vi "Measurement UI.vi"() -> ()   [LabVIEW 2022 SP3, in "Efficiency_Class D Amplifier_UI.lvlib"]
uses:
  Efficiency_Class D Amplifier_UI.lvlib
  shared/controls/units - snr.ctl
  shared/controls/units - ratio.ctl
  shared/controls/digital output level units.ctl
  shared/ui/controls/view.ctl
  shared/controls/power measurement method.ctl
  UI State.ctl
  <vilib>/Utility/miscctls.llb/LVBoundsTypeDef.ctl
  <vilib>/Utility/miscctls.llb/LVPoint32TypeDef.ctl
  <vilib>/Utility/miscctls.llb/LVPointTypeDef.ctl
  shared/ui/UI Helpers.lvlib
  shared/audio popup ui/Audio Popup UI.lvlib
  shared/controls/audio controls.lvlib
panel:
  in  "view legend":T1
  out "time domain":waveform(dbl)[](graph)
  out "frequency domain":cluster{"x0":dbl, "dx":dbl, "magnitude":dbl[]}[](graph)
  out "efficiency (%)":dbl caption="Efficiency" format="%#.2g%"
  out "power loss (W)":dbl caption="Power Loss" format="%#.2g W"
  out "total output power (W)":dbl caption="Total Output Power" format="%#.2g W"
  out "input power (W)":dbl caption="Input Power" format="%#.2g W"
  out "meas table":string[][](table)
  in  "digital serial cfg file":string
  in  "power measurement resource":string="PXI1Slot4/ai0"
  out "output power (W)":dbl[](array[numeric])
  out "SFDR (dBc)":dbl[](array[numeric])
  out "gain":dbl[](array[numeric])
  out "dynamic range (dB)":dbl[](array[numeric])
  out "THD":dbl[](array[numeric])
  out "THD+N":dbl[](array[numeric])
  out "SNR":dbl[](array[numeric])
  out "phase (deg)":dbl[](array[numeric])
  out "amplitude (dBFS)":dbl[](array[numeric])
  out "amplitude (Vrms)":dbl[](array[numeric])
  out "frequency (Hz)":dbl[](array[numeric])
  out "channel names":string[](array[string])
  in  "Configuration tab":enum32{"Protocol", "Measurement", "Units"}(tab)
  out "digital serial file name":string
  in  "configure digital serial":bool
  in  "master clock channel list":string caption="Master Clock Channel"
  in  "digital channel list":string caption="Digital Audio Channel"
  in  "sense resistor (Ohms)":dbl caption="Sense Resistor" format="%#_g Ohms"
  in  "power supply current limit":dbl caption="Current Limit" format="%#_g A"
  in  "power supply voltage":dbl caption="Power Supply Voltage" format="%#_g V"
  in  "power meas resource":refnum<k15> caption="Resource"
  in  "power measurement method":T2 caption="Method"
  in  "output level":dbl=-1.0 caption="Output level" format="%#_3f"
  in  "output level units":T3
  in  "min settling cycles":u32 caption="Minimum settling cycles"
  in  "min settling time (s)":dbl=0.1 caption="Minimum settling time" format="%#_6ps"
  in  "min measurement cycles":u32 caption="Minimum measurement cycles"
  in  "min measurement time (s)":dbl=0.1 caption="Minimum measurement time" format="%#_6ps"
  in  "Acquisition channel":tag
  in  "acq sampling rate":dbl=51200.0 caption="Sample rate" format="%#.6pHz"
  in  "lowpass filter":T4(ring) caption="Lowpass filter"
  in  "highpass filter":enum32{"DC", "AC"}(ring) caption="Highpass filter"
  in  "band start":dbl=20.0 caption="Band start" format="%#_6pHz"
  in  "band stop":dbl=20000.0 caption="Band stop" format="%#_6pHz"
  in  "weighting filter":T5(ring)=enum."A-weighting" caption="Weighting filter"
  in  "load impedance":dbl=4.0 caption="Load impedance" format="%#_6p Ohms"
  in  "output range (pk-pk)":dbl=15.0 caption="Output range" format="%.3p Vpk-pk"
  in  "signal frequency":dbl=1000.0 caption="Frequency" format="%#_6pHz"
  in  "gain units":T6 caption="Gain"
  in  "THD units":T6 caption="THD"
  in  "THD+N units":T6 caption="THD+N"
  in  "SNR units":T7 caption="SNR"
  in  "channel 0 offset":u32=1
  out "fft - data":dbl[](array[numeric])
  out "fft - df":dbl
  out "fft - f0":dbl
  out "wfm - data":dbl[](array[numeric])
  out "wfm - dt":dbl
  out "wfm - t0":dbl
  in  "acq channel":string="PXI1Slot4/ai0"
  in  "signal phase":dbl caption="phase"
  # "hidden controls - used to sync with MeasLink"
  # "hidden indicators"
  # "Digital Serial Settings"
  # "Harware Resource"
  # "Filters"
  # "Output"
  # "Acquisition"
  # "Power"
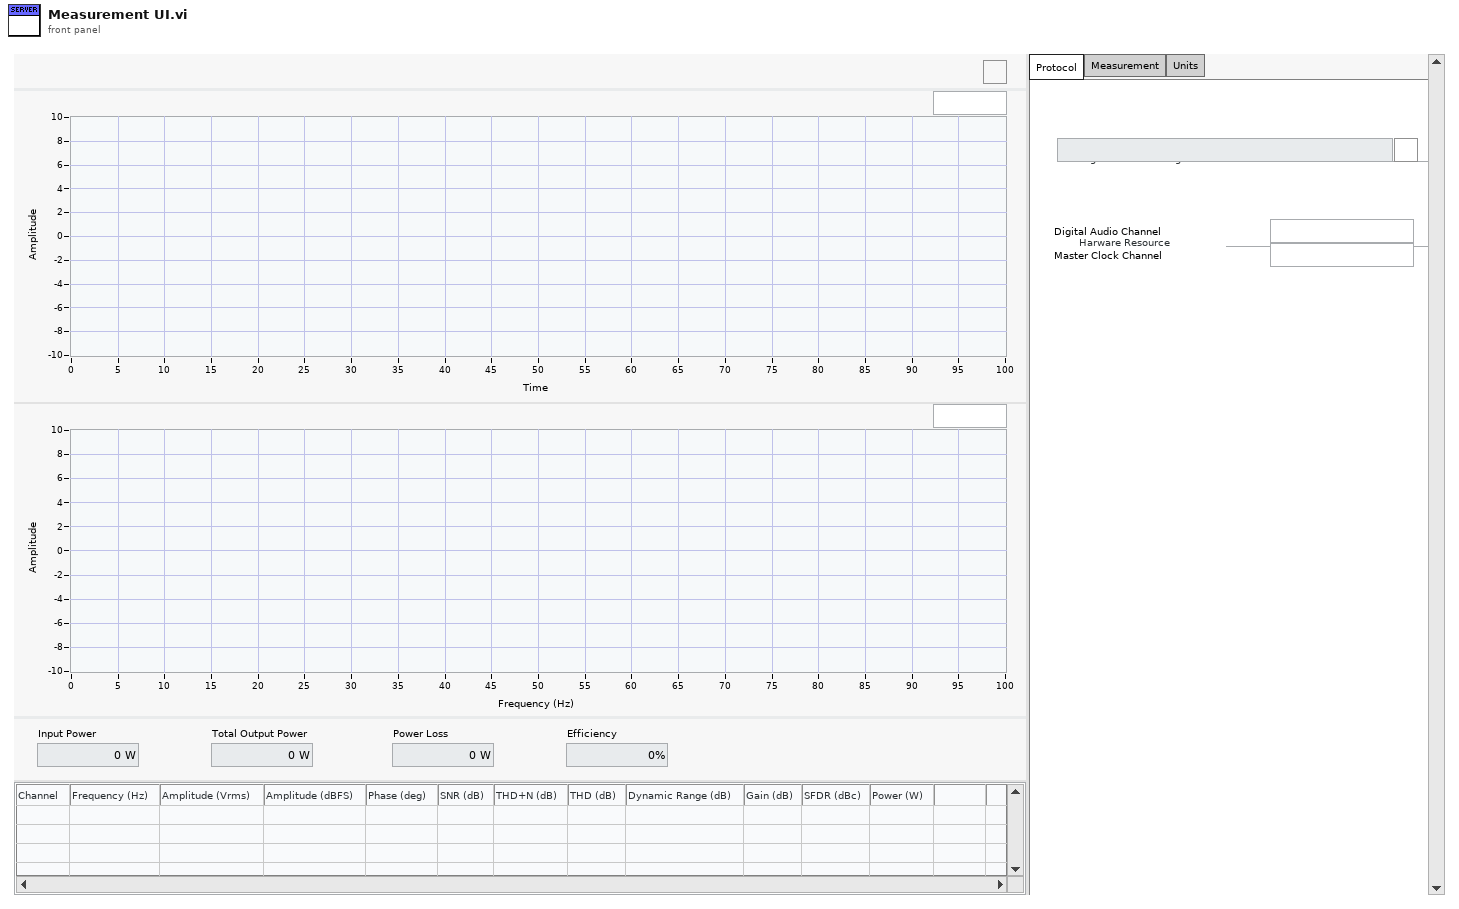
[diagram p1: front panel]
types:
  T1 = typedef "UI Helpers.lvlib/view.ctl" = bool
  T2 = typedef "power measurement method.ctl" = enum32{"SMU", "DMM"}
  T3 = typedef "audio controls.lvlib/digital output level units.ctl" = enum32{"% FS", "dBFS", "V"}
  T4 = enum32{"No filter", "AES17 20kHz", "AES17 40kHz"}
  T5 = enum32{"Linear", "A-weighting", "B-weighting", "C-weighting"}
  T6 = typedef "audio controls.lvlib/units - ratio.ctl" = enum32{"dB", "%", "x/y"}
  T7 = typedef "audio controls.lvlib/units - snr.ctl" = enum32{"dB", "x/y"}
  T8 = typedef "Efficiency_Class D Amplifier_UI.lvlib/UI State.ctl" = cluster{"Graph Size":T9, "Legend Visible":bool, "Mouse Coords":T10, "PostUI event occurred":bool, "digital serial cfg file":path}
  T9 = typedef "LVBoundsTypeDef.ctl" = cluster{"Width":u32, "Height":u32}
  T10 = typedef "LVPoint32TypeDef.ctl" = cluster{"Horizontal":i32, "Vertical":i32}
  T11 = typedef "LVPointTypeDef.ctl" = cluster{"Horizontal":i16, "Vertical":i16}
  T12 = typedef "Audio Popup UI.lvlib/audio settings.ctl" = cluster{"digital serial file":string}
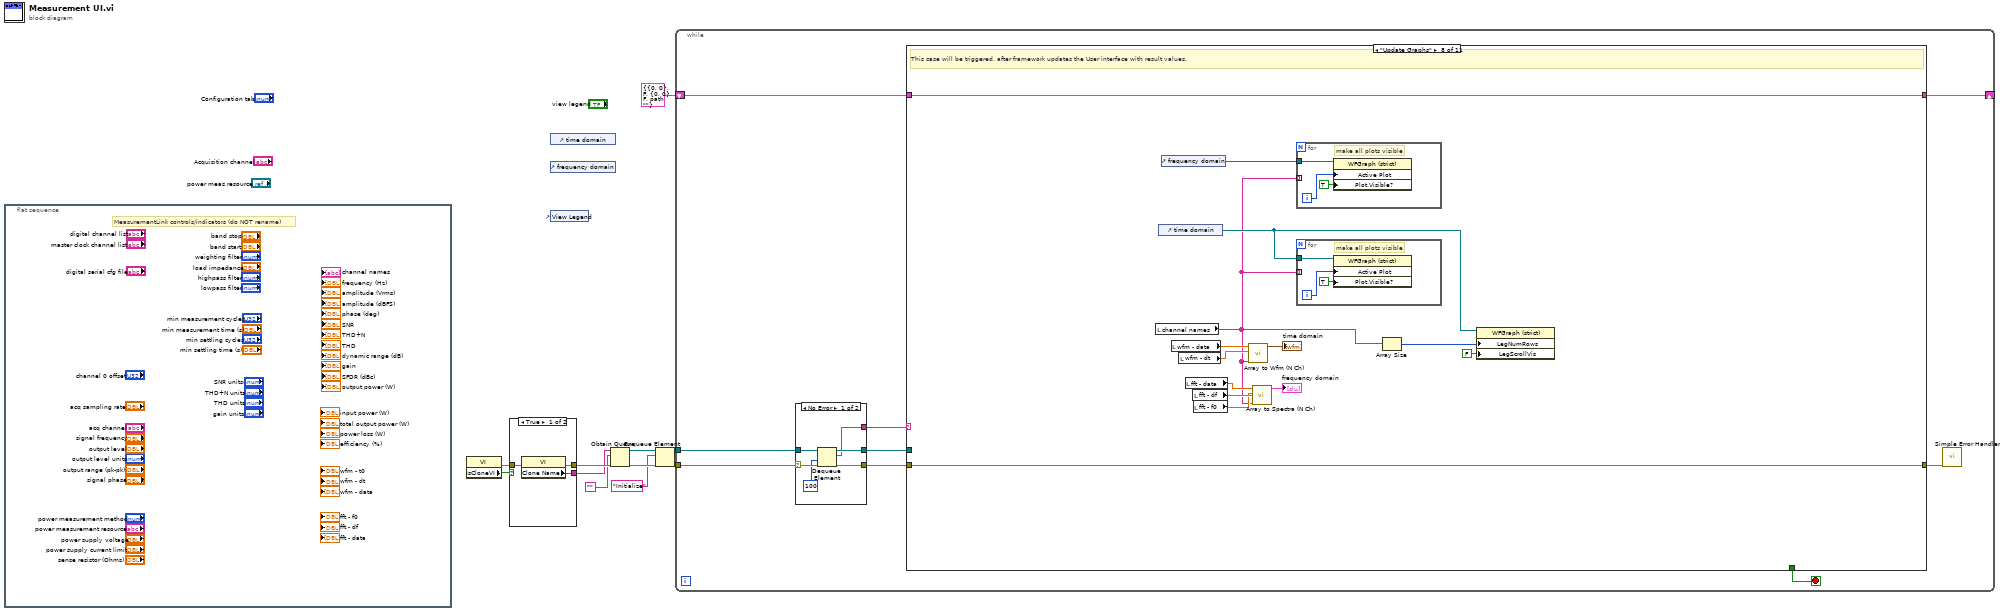
[diagram p0: block diagram]
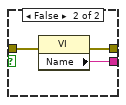
[diagram p2: hidden frame]
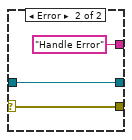
[diagram p3: hidden frame]
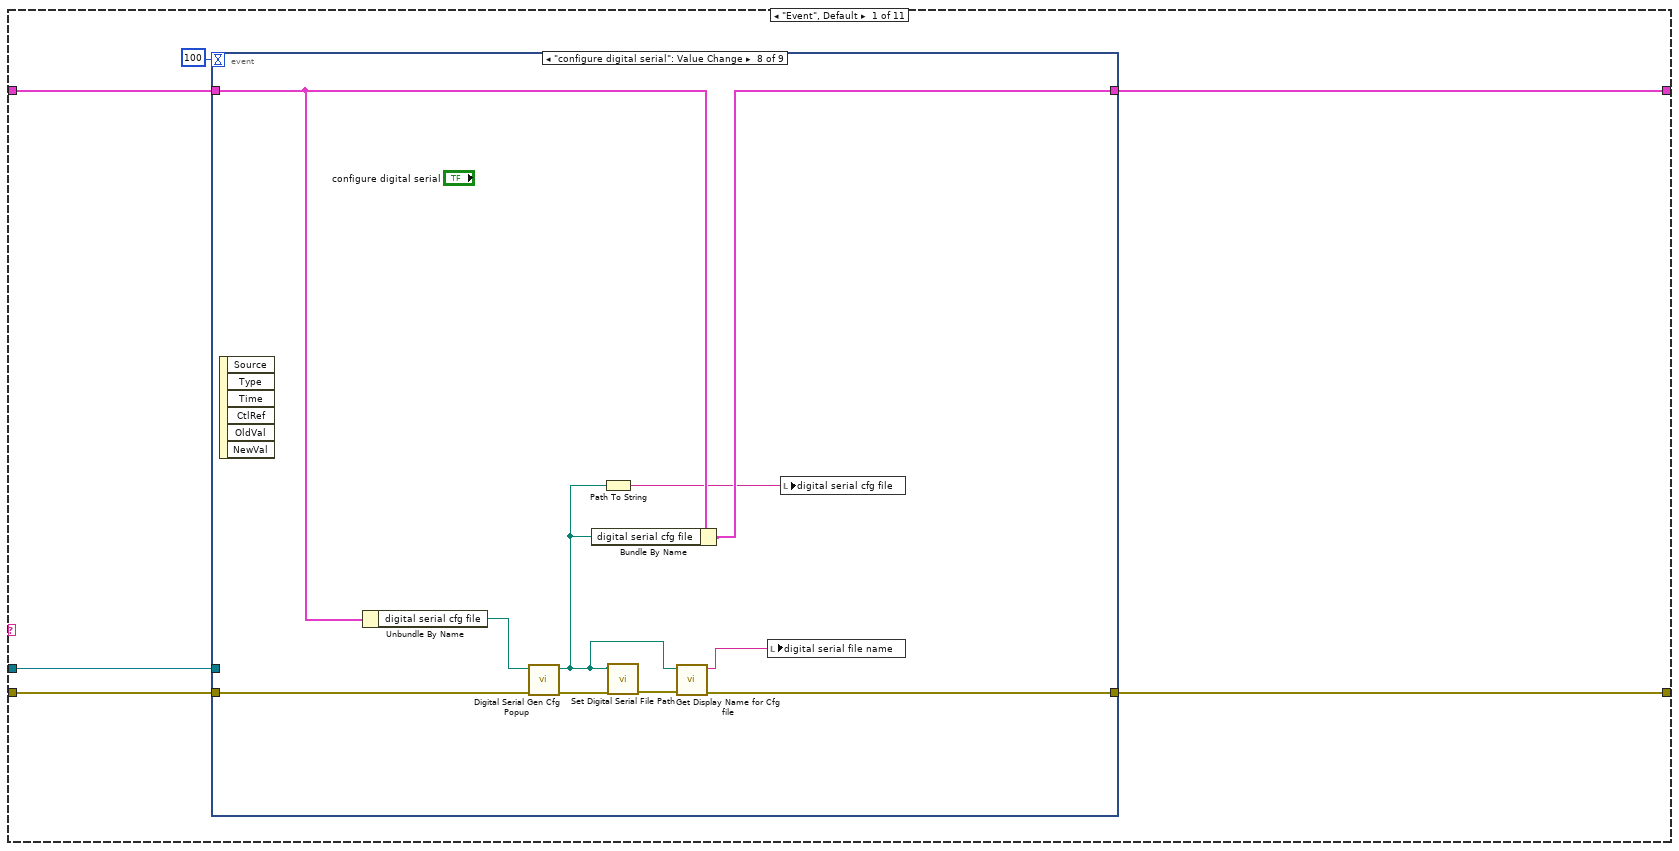
[diagram p4: hidden frame]
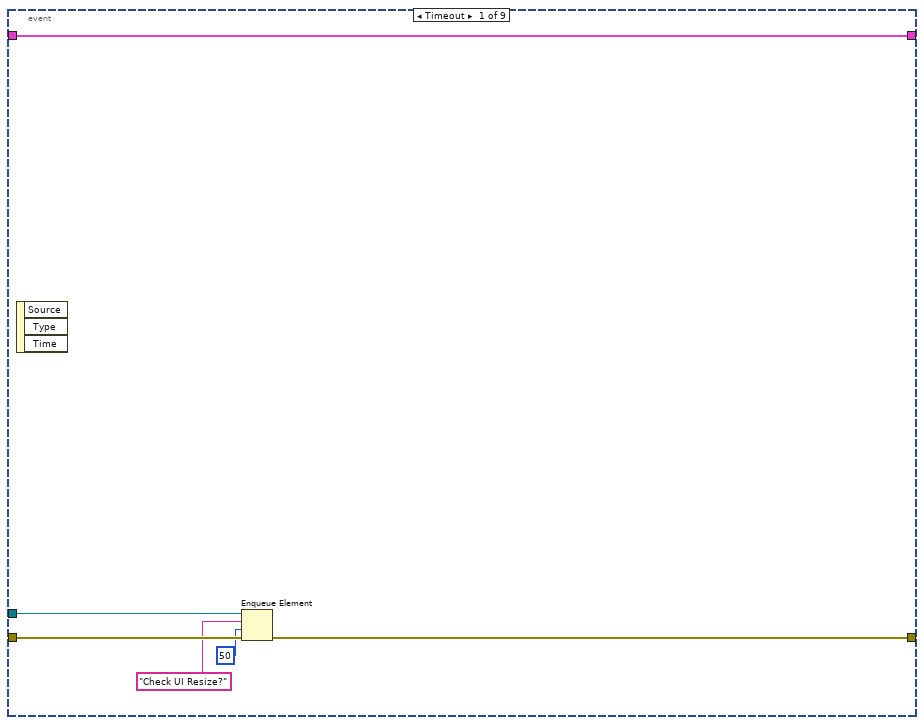
[diagram p5: hidden frame]
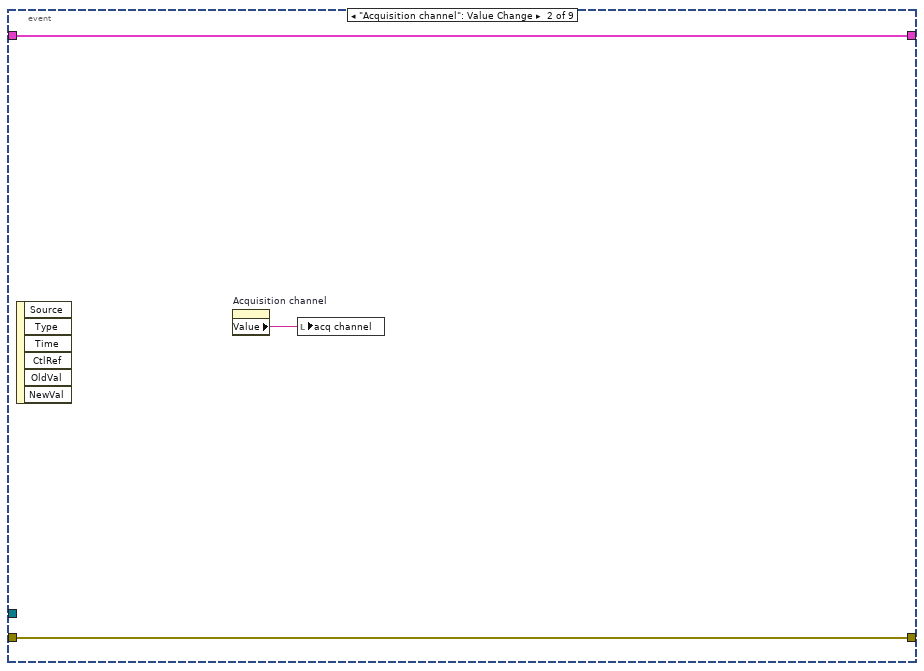
[diagram p6: hidden frame]
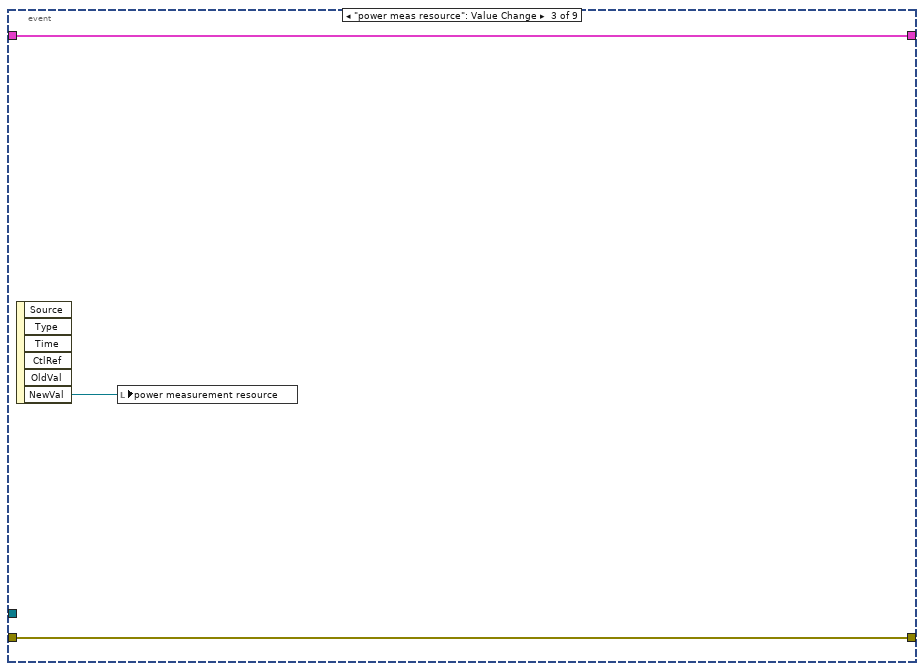
[diagram p7: hidden frame]
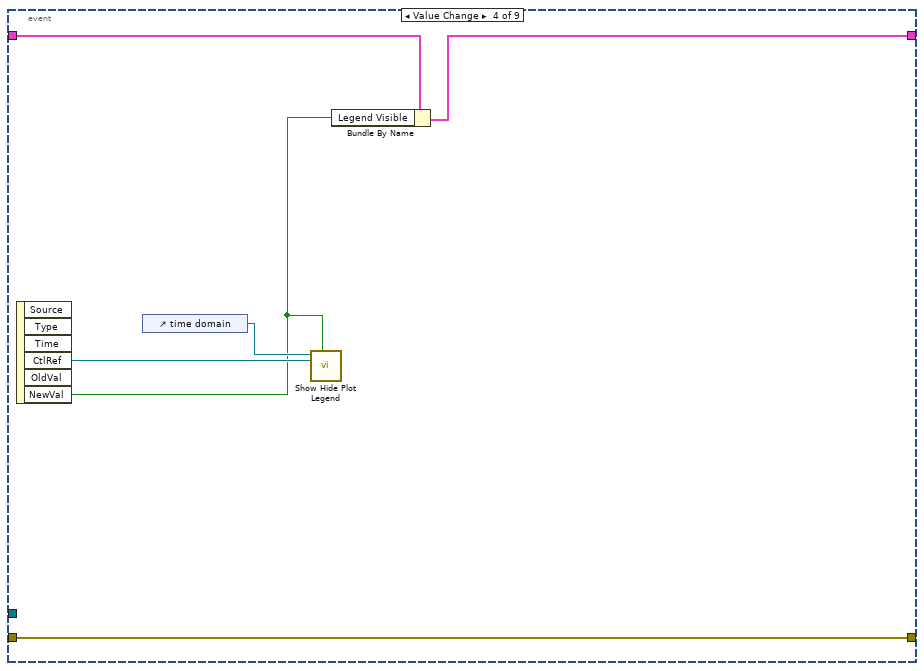
[diagram p8: hidden frame]
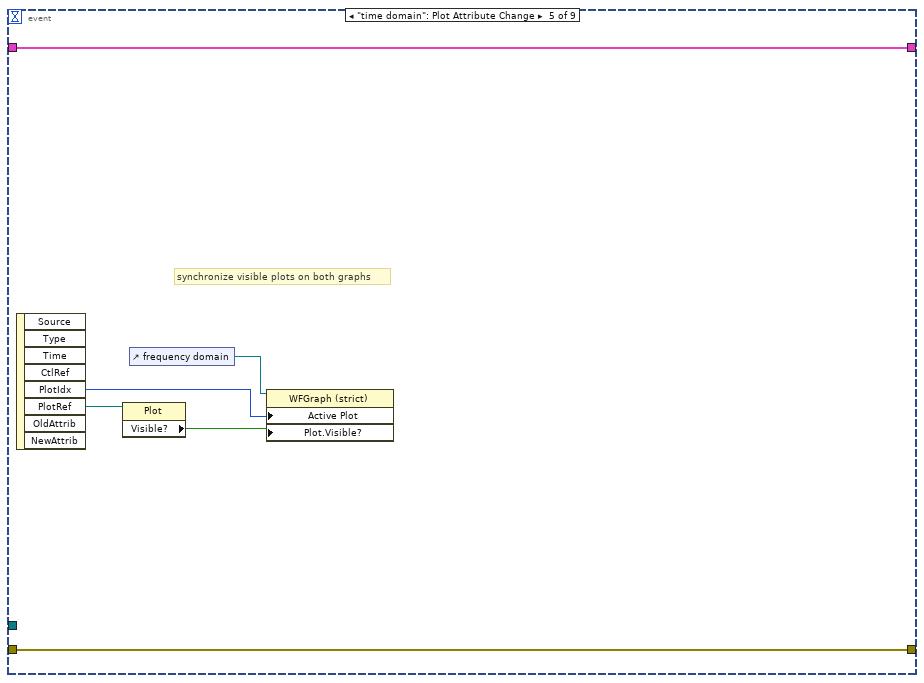
[diagram p9: hidden frame]
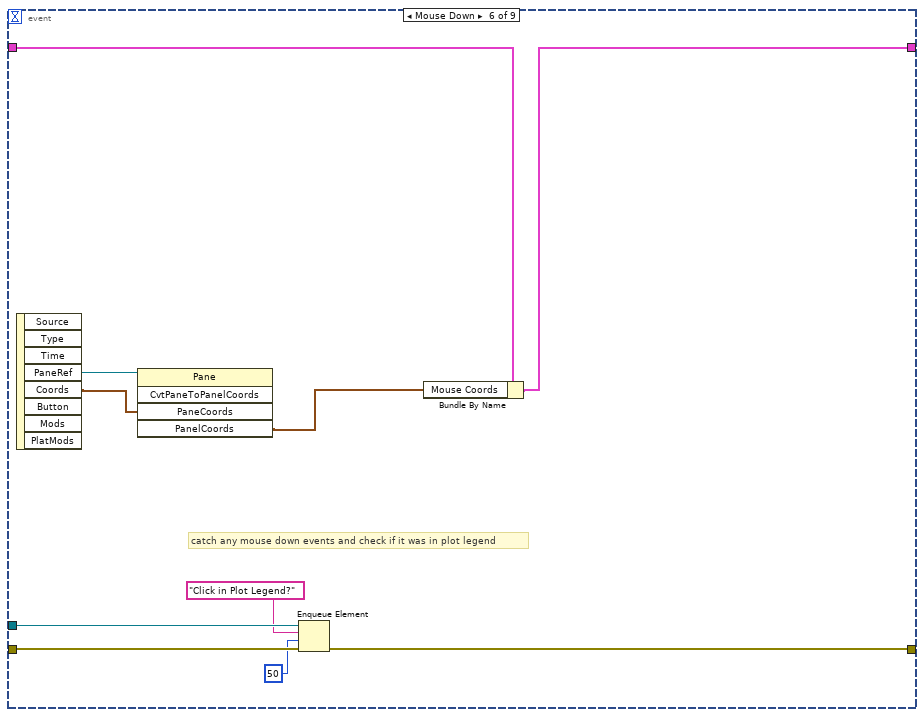
[diagram p10: hidden frame]
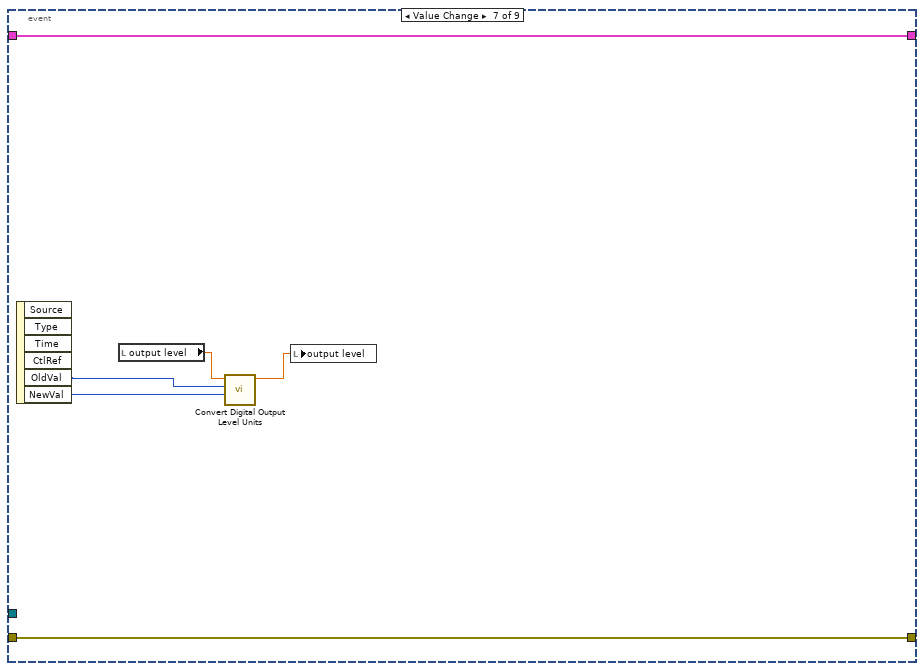
[diagram p11: hidden frame]
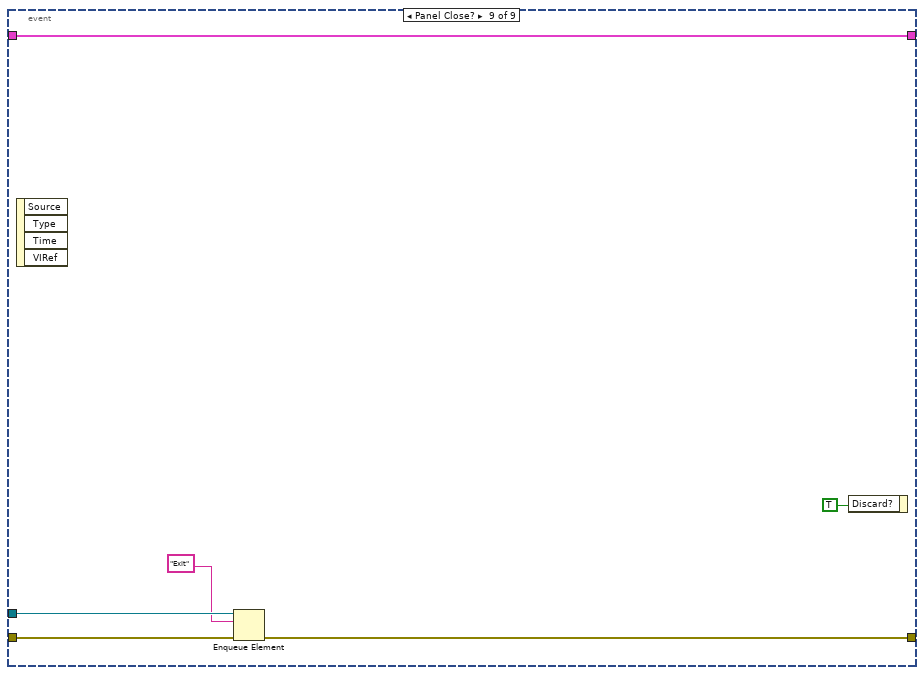
[diagram p12: hidden frame]
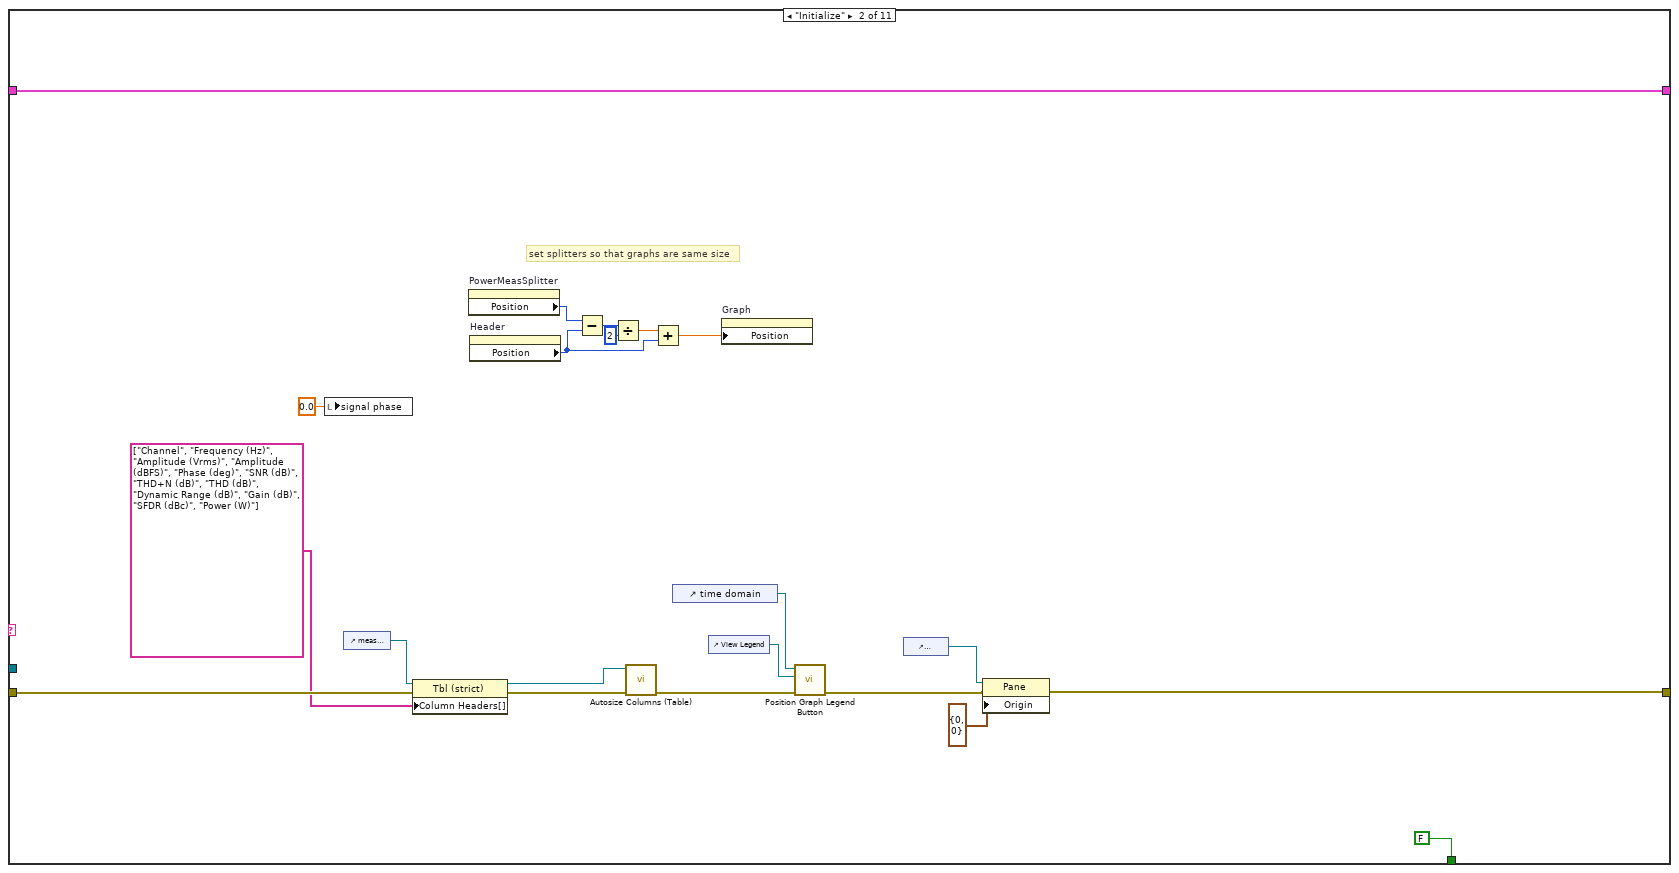
[diagram p13: hidden frame]
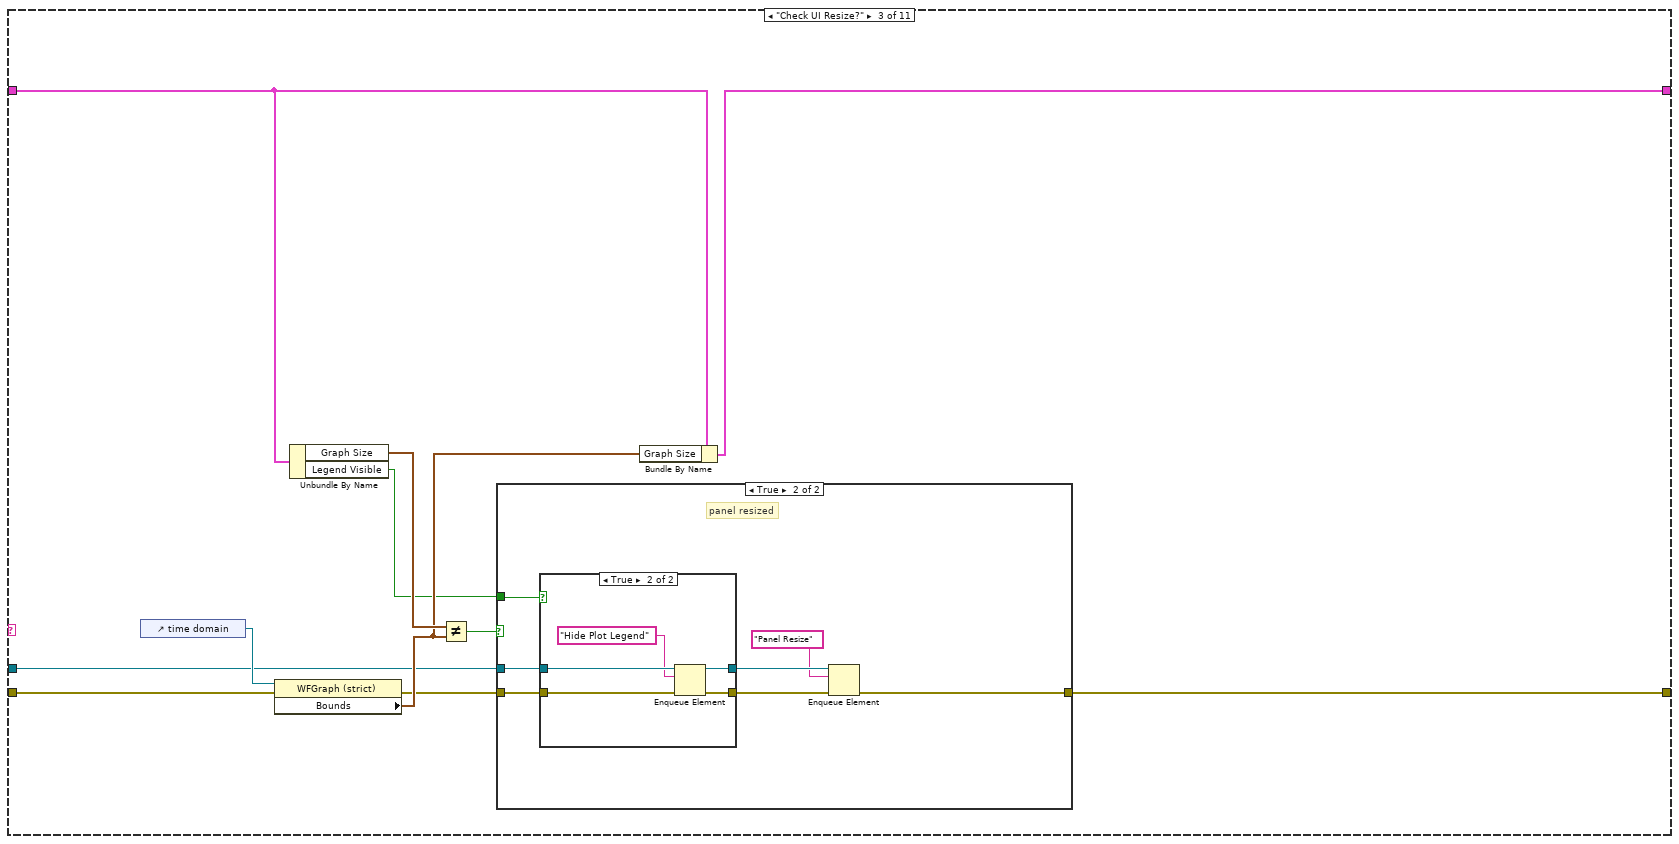
[diagram p14: hidden frame]
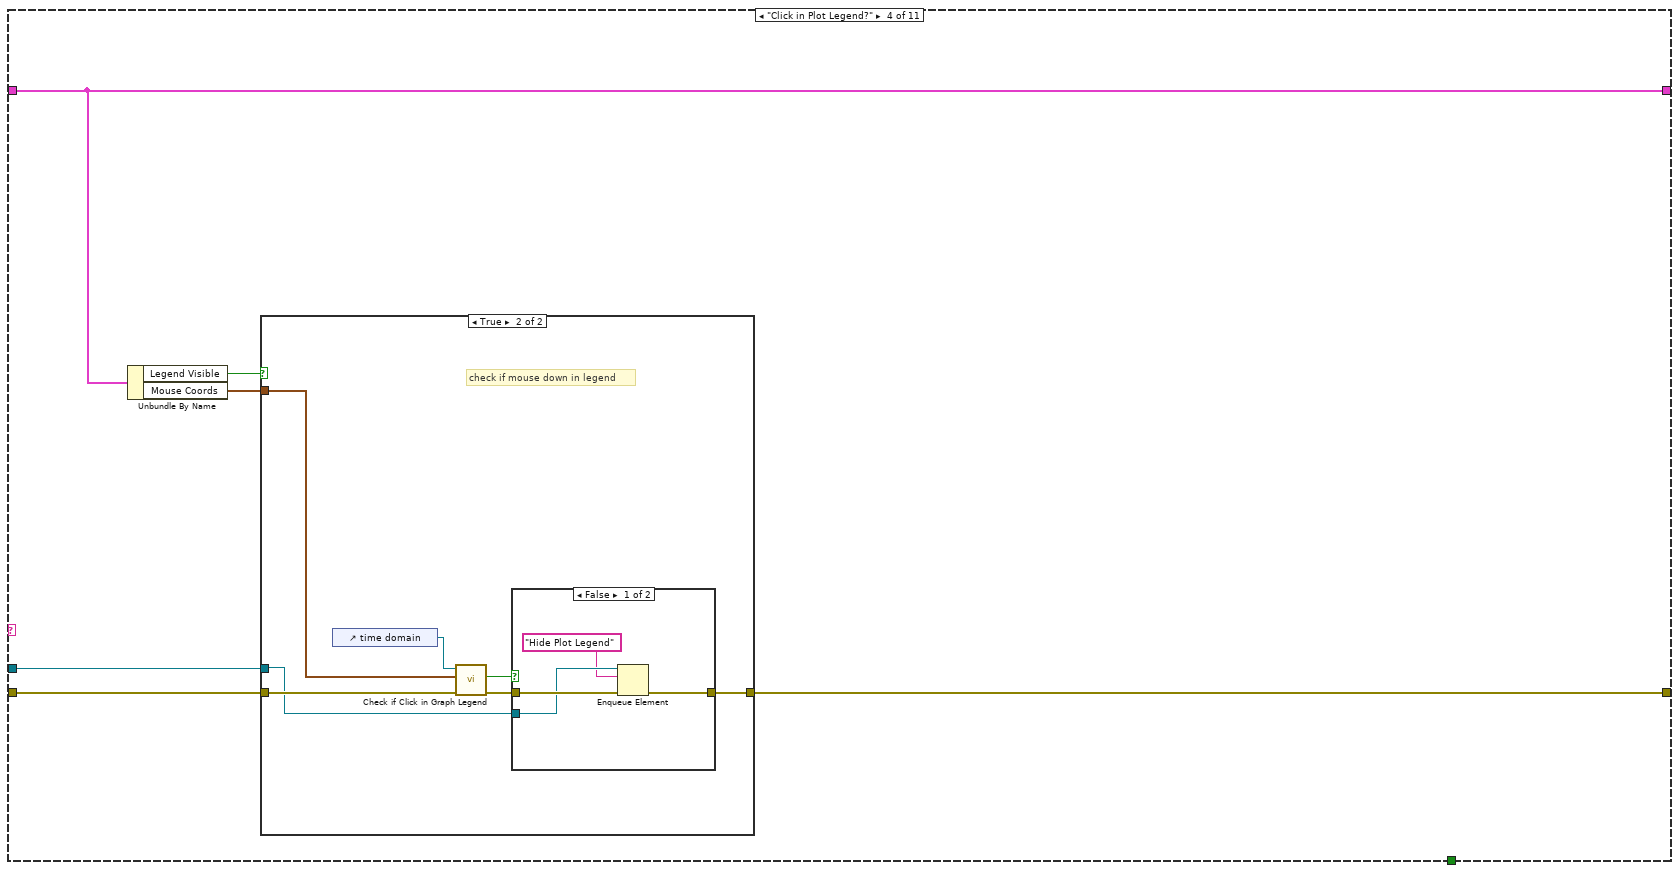
[diagram p17: hidden frame]
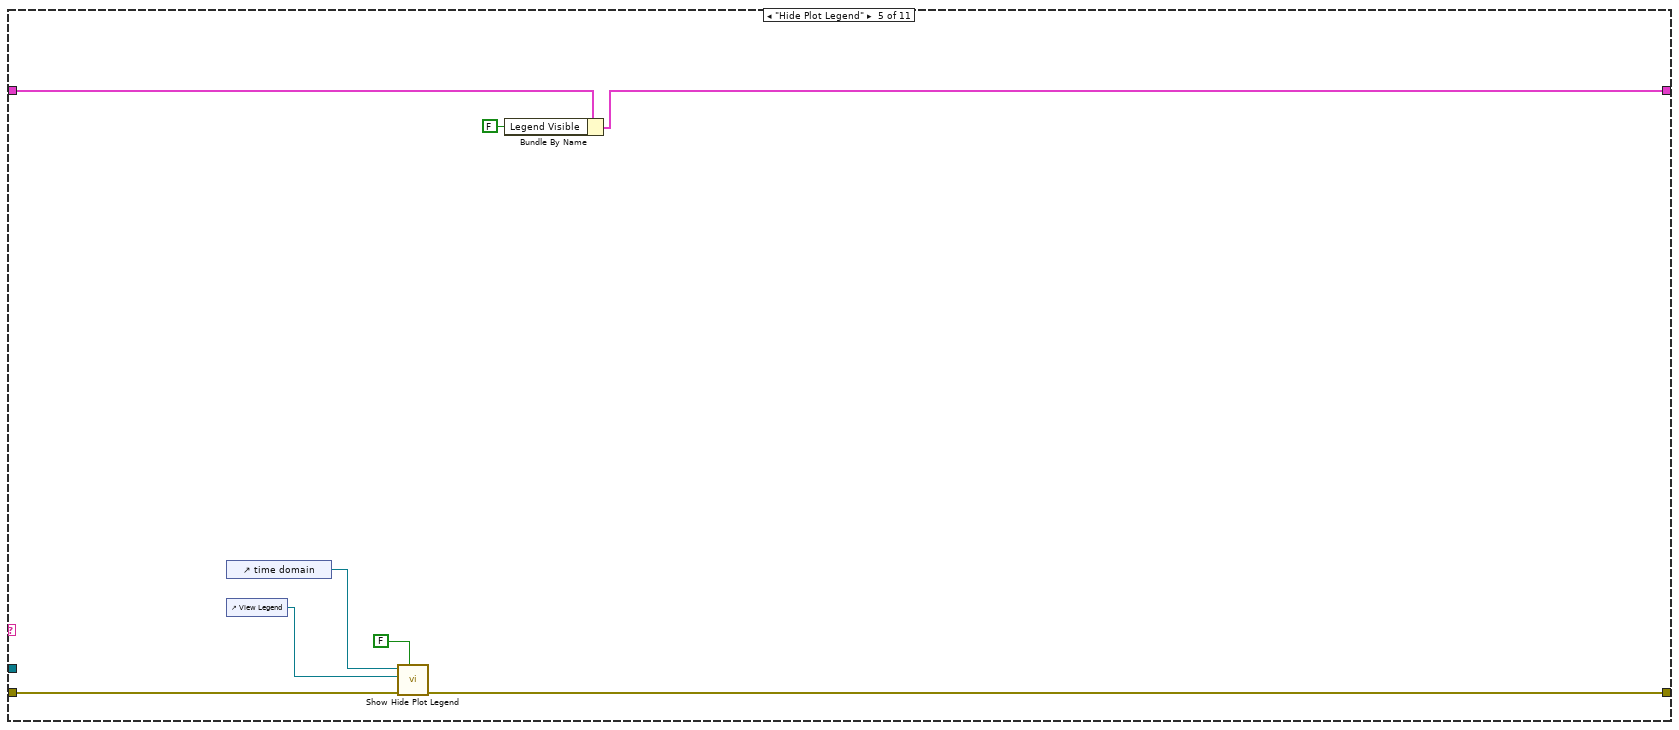
[diagram p20: hidden frame]
diagram:
  n1 = flat-sequence {
    frame #0 {
      # "MeasurementLink controls/indicators (do NOT rename)"
    }
  }
  n2 = property class="VI"() -> (error out=w2:errorcluster, "IsCloneVI"=w3:bool)  [unwired: 2 in, 1 out]
  n3 = case shown="True" w3 {
    tunnel: [w14 w17] -> w11
    tunnel: [w13 w16] -> w10
    tunnel: w2 -> [w12 w15]
    frame True {
      n4 = property class="VI"(error in=w12) -> (error out=w14:errorcluster, "Clone Name"=w13:string)  [unwired: 1 in, 1 out]
    }
    frame False {
      n5 = property class="VI"(error in=w15) -> (error out=w17:errorcluster, "Name"=w16:string)  [unwired: 1 in, 1 out]
    }
  }
  n6 = control-ref of="time domain"() -> ()  [unwired: 1 out]
  n7 = control-ref of="frequency domain"() -> ()  [unwired: 1 out]
  n8 = control-ref of="View Legend"() -> ()  [unwired: 1 out]
  n9 = Obtain Queue(name (unnamed)=w10, element data type="", error in (no error)=w11) -> (queue out=w7:refnum<queue>, error out=w9:errorcluster)  [unwired: 2 in, 1 out]
  n10 = Enqueue Element(queue=w7, element="Initialize", error in (no error)=w9) -> (queue out=w6:refnum<queue>, error out=w8:errorcluster)  [unwired: 1 in, 1 out]
  n11 = while {
    tunnel: w6 -> [w24]
    shift-right: [w20] -> _
    shift-left: T8 {"Graph Size"={"Width"=0, "Height"=0}, "Legend Visible"=FALSE, "Mouse Coords"={"Horizontal"=0, "Vertical"=0}, "PostUI event occurred"=FALSE, "digital serial cfg file"=path ""} ("ui state") -> [w19]
    tunnel: w8 -> [w26]
    stop <- w21 stop-if-true
    n12 = case shown="No Error" w26 {
      selector: w26 -> [w32 w35]
      tunnel: [w31 w35] -> w25
      tunnel: w24 -> [w30 w34]
      tunnel: [w29 w34] -> w23
      tunnel: [w28 "Handle Error"] -> w22
      frame No Error {
        n13 = Dequeue Element(queue=w30, timeout in ms (-1)=100, error in (no error)=w32) -> (queue out=w29:refnum<queue>, element=w28:string, error out=w31:errorcluster)  [unwired: 1 out]
      }
      frame Error {
      }
    }
    n14 = case shown="\"Update Graphs\"" w22 {
      tunnel: w25 -> [w40 w113 w128 w146 w168 w173 w184 w223 w231 w357 w359]
      tunnel: w23 -> [w38 _ w119 w147 _ _ w183 _ _ w355 _]
      tunnel: [w41 w101 w121 w145 w167 w172 w179 w223 w235 w352 w359] -> w18
      tunnel: [_ FALSE _ _ _ _ _ _ _ TRUE _] -> w21
      tunnel: [w36 w98 w124 w150 w169 w176 w177 w224 w232 w350 w358] -> w20
      tunnel: w19 -> [w37 w98 w125 w150 w170 w176 w178 w224 w232 w350 w358]
      frame "Event", Default {
        n15 = event shown="[7] \"configure digital serial\": Value Change" {
          selector: _ -> [_ _ _ _ _ _ _ _ _]
          dyn-events: _ -> [_ _ _ _ _ _ _ _ _]
          timeout: 100 -> [_ _ _ _ _ _ _ _ _]
          tunnel: [w44 w48 w53 w56 w60 w73 w76 w86 w95] -> w41
          tunnel: w40 -> [w47 w48 w53 w56 w60 w74 w76 w87 w96]
          tunnel: w38 -> [w46 _ _ _ _ w75 _ _ w94]
          tunnel: w37 -> [w43 w49 w52 w58 w61 w70 w77 w85 w92]
          tunnel: [w43 w49 w52 w57 w61 w69 w77 w84 w92] -> w36
          event Timeout {
            n16 = event-data() -> ()  [unwired: 1 in, 3 out]
            n17 = Enqueue Element(queue=w46, element="Check UI Resize?", timeout in ms (-1)=50, error in (no error)=w47) -> (error out=w44:errorcluster)  [unwired: 2 out]
          }
          event "Acquisition channel": Value Change {
            n18 = event-data() -> ()  [unwired: 1 in, 6 out]
            n19 = property on="Acquisition channel" class="DAQmxName"() -> ("Value"=w50:string)  [unwired: 2 in, 2 out]
            n20 = local write "acq channel"(w50) -> ()
          }
          event "power meas resource": Value Change {
            n21 = event-data() -> ("NewVal"=w51:refnum<k15>)  [unwired: 1 in, 5 out]
            n22 = local write "power measurement resource"(w51) -> ()
          }
          event Value Change {
            n23 = event-data() -> ("CtlRef"=w55:refnum<vi>, "NewVal"=w54:T1)  [unwired: 1 in, 4 out]
            n24 = control-ref of="time domain"() -> (w59:refnum<vi>)
            n25 = call "Show Hide Plot Legend.vi"("show"=w54, "view reference"=w55, "graph reference"=w59) -> ()  [unwired: 8 in, 1 out]
            n26 = Bundle By Name(cluster=w58, "Legend Visible"=w54) -> (w57:T8)
          }
          event "time domain": Plot Attribute Change {
            # "synchronize visible plots on both graphs"
            n27 = event-data() -> ("PlotIdx"=w63:i32, "PlotRef"=w64:refnum<vi>)  [unwired: 1 in, 6 out]
            n28 = property class="Plot"(reference=w64) -> ("Visible?"=w65:bool)  [unwired: 1 in, 2 out]
            n29 = control-ref of="frequency domain"() -> (w62:refnum<vi>)
            n30 = property on="Property Node" class="WFGraph (strict)"(reference=w62, "Active Plot"=w63, "Plot.Visible?"=w65) -> ()  [unwired: 1 in, 2 out]
          }
          event Mouse Down {
            # "catch any mouse down events and check if it was in plot legend"
            n31 = event-data() -> ("PaneRef"=w68:refnum<vi>, "Coords"=w67:T10)  [unwired: 1 in, 6 out]
            n32 = invoke class="Pane" method="CvtPaneToPanelCoords"(reference=w68, "PaneCoords"=w67) -> ("PanelCoords"=w66:T11)  [unwired: 3 in, 4 out]
            n33 = Enqueue Element(queue=w75, element="Click in Plot Legend?", timeout in ms (-1)=50, error in (no error)=w74) -> (error out=w73:errorcluster)  [unwired: 2 out]
            n34 = Bundle By Name(cluster=w70, "Mouse Coords"=w66) -> (w69:T8)
          }
          event Value Change {
            n35 = event-data() -> ("OldVal"=w81:T3, "NewVal"=w80:T3)  [unwired: 1 in, 4 out]
            n36 = local read "output level"() -> (w79:dbl)
            n37 = call "Convert Digital Output Level Units.vi"("new output level units"=w80, "previous output level units"=w81, "previous output level"=w79) -> ("new output level"=w78:dbl)  [unwired: 8 in]
            n38 = local write "output level"(w78) -> ()
          }
          event "configure digital serial": Value Change {
            n39 = event-data() -> ()  [unwired: 1 in, 6 out]
            n40 = Unbundle By Name(w85) -> ("digital serial cfg file"=w91:path)
            n41 = call "Digital Serial Gen Cfg Popup.vi"("error in (no error)"=w87, "config file in"=w91) -> ("error out"=w90:errorcluster, "config file out"=w88:path)  [unwired: 7 in, 1 out]
            n42 = Bundle By Name(cluster=w85, "digital serial cfg file"=w88) -> (w84:T8)
            n43 = Path To String(path=w88) -> (string=w83:string)
            n44 = call "Set Digital Serial File Path.vi"("error in (no error)"=w90, "digital serial file"=w88) -> ("error out"=w89:errorcluster)  [unwired: 9 in]
            n45 = call "Get Display Name for Cfg file.vi"("error in (no error)"=w89, "file path"=w88) -> ("error out"=w86:errorcluster, "display string"=w82:string)  [unwired: 8 in]
            n46 = local write "digital serial file name"(w82) -> ()
            n47 = local write "digital serial cfg file"(w83) -> ()
          }
          event Panel Close? {
            n48 = event-data() -> ()  [unwired: 1 in, 4 out]
            n49 = Enqueue Element(queue=w94, element="Exit", error in (no error)=w96) -> (error out=w95:errorcluster)  [unwired: 1 in, 2 out]
            n50 = event-data("Discard?"=TRUE) -> ()  [unwired: 1 in, 1 out]
          }
        }
      }
      frame "Initialize" {
        # "set splitters so that graphs are same size"
        n51 = local write "signal phase"(0.0 ("signal phase")) -> ()
        n52 = control-ref of="meas table"() -> (w111:refnum<vi>)
        n53 = property class="Tbl (strict)"(reference=w111, error in=w113, "Column Headers[]"=string[] ["Channel", "Frequency (Hz)", "Amplitude (Vrms)", "Amplitude (dBFS)", "Phase (deg)", "SNR (dB)", "THD+N (dB)", "THD (dB)", "Dynamic Range (dB)", "Gain (dB)", "SFDR (dBc)", "Power (W)"] ("Column Header Strings[]")) -> (reference out=w110:refnum<vi>, error out=w112:errorcluster)
        n54 = property on="PowerMeasSplitter" class="Splitter"() -> ("Position"=w108:i32)  [unwired: 2 in, 2 out]
        n55 = property on="Header" class="Splitter"() -> ("Position"=w104:i32)  [unwired: 2 in, 2 out]
        n56 = Subtract(x=w108, y=w104) -> (x-y=w107:i32)
        n57 = Divide(x=w107, y=2) -> (x/y=w105:dbl)
        n58 = call "Autosize Columns (Table).vi"("error in (no error)"=w112, "table"=w110) -> ("error out"=w114:errorcluster)  [unwired: 9 in]
        n59 = Add(x=w105, y=w104) -> (x+y=w103:dbl)
        n60 = control-ref of="time domain"() -> (w116:refnum<vi>)
        n61 = control-ref of="View Legend"() -> (w115:refnum<vi>)
        n62 = property on="Graph" class="Splitter"("Position"=w103) -> ()  [unwired: 2 in, 2 out]
        n63 = call "Position Graph Legend Button.vi"("error in (no error)"=w114, "view legend"=w115, "graph"=w116) -> ("error out"=w102:errorcluster)  [unwired: 8 in]
        n64 = control-ref of="Configuration"() -> (w100:refnum<vi>)
        n65 = property class="Pane"(reference=w100, error in=w102, "Origin"=T11 {"Horizontal"=0, "Vertical"=0}) -> (error out=w101:errorcluster)  [unwired: 1 out]
      }
      frame "Check UI Resize?" {
        n66 = control-ref of="time domain"() -> (w129:refnum<vi>)
        n67 = property on="Property Node" class="WFGraph (strict)"(reference=w129, error in=w128) -> (error out=w122:errorcluster, "Bounds"=w126:T9)  [unwired: 1 out]
        n68 = Unbundle By Name(w125) -> ("Graph Size"=w127:T9, "Legend Visible"=w120:bool)
        n69 = Not Equal?(x=w127, y=w126) -> (x != y?=w123:bool)
        n70 = case shown="True" w123 {
          tunnel: w122 -> [w130 w137]
          tunnel: [w130 w132] -> w121
          tunnel: w120 -> [_ w135]
          tunnel: w119 -> [_ w136]
          frame False {
            # "no resize"
          }
          frame True {
            # "panel resized"
            n71 = case shown="True" w135 {
              tunnel: w137 -> [w139 w144]
              tunnel: [w139 w143] -> w134
              tunnel: w136 -> [w138 w142]
              tunnel: [w138 w140] -> w133
              frame False {
              }
              frame True {
                n72 = Enqueue Element(queue=w142, element="Hide Plot Legend", error in (no error)=w144) -> (queue out=w140:refnum<queue>, error out=w143:errorcluster)  [unwired: 1 in, 1 out]
              }
            }
            n73 = Enqueue Element(queue=w133, element="Panel Resize", error in (no error)=w134) -> (error out=w132:errorcluster)  [unwired: 1 in, 2 out]
          }
        }
        n74 = Bundle By Name(cluster=w125, "Graph Size"=w126) -> (w124:T8)
      }
      frame "Click in Plot Legend?" {
        n75 = Unbundle By Name(w150) -> ("Legend Visible"=w149:bool, "Mouse Coords"=w148:T10)
        n76 = case shown="True" w149 {
          tunnel: w148 -> [_ w156]
          tunnel: w147 -> [_ w153]
          tunnel: w146 -> [w151 w158]
          tunnel: [w151 w152] -> w145
          frame False {
            # "legend not visible; do nothing"
          }
          frame True {
            # "check if mouse down in legend"
            n77 = control-ref of="time domain"() -> (w157:refnum<vi>)
            n78 = call "Check if Click in Graph Legend.vi"("error in (no error)"=w158, "Mouse Coords"=w156, "WaveformGraph"=w157) -> ("error out"=w154:errorcluster, "click in legend?"=w155:bool)  [unwired: 7 in]
            n79 = case shown="False" w155 {
              tunnel: w154 -> [w162 w163]
              tunnel: w153 -> [w161 _]
              tunnel: [w160 w163] -> w152
              frame False {
                n80 = Enqueue Element(queue=w161, element="Hide Plot Legend", error in (no error)=w162) -> (error out=w160:errorcluster)  [unwired: 1 in, 2 out]
              }
              frame True {
                # "inside legend; do nothing"
              }
            }
          }
        }
      }
      frame "Hide Plot Legend" {
        n81 = control-ref of="time domain"() -> (w165:refnum<vi>)
        n82 = control-ref of="View Legend"() -> (w164:refnum<vi>)
        n83 = call "Show Hide Plot Legend.vi"("show"=FALSE, "error in (no error)"=w168, "view reference"=w164, "graph reference"=w165) -> ("error out"=w167:errorcluster)  [unwired: 7 in]
        n84 = Bundle By Name(cluster=w170, "Legend Visible"=FALSE ("legend visible")) -> (w169:T8)
      }
      frame "Panel Resize" {
        n85 = control-ref of="time domain"() -> (w175:refnum<vi>)
        n86 = control-ref of="View Legend"() -> (w174:refnum<vi>)
        n87 = call "Position Graph Legend Button.vi"("error in (no error)"=w173, "view legend"=w174, "graph"=w175) -> ("error out"=w172:errorcluster)  [unwired: 8 in]
      }
      frame "Post UI Update" {
        # "This case will be triggered, after framework updates the User interface with result values."
        n88 = Unbundle By Name(w178) -> ("PostUI event occurred"=w181:bool)
        n89 = for {
          tunnel: w183 -> [w208]
          shift-right: [w207] -> w180
          shift-left: w184 -> [w209]
          tunnel: string[] ["Update Table", "Update Graphs"] -> [w206] mode=indexing
          n90 = Enqueue Element(queue=w208, element=w206, timeout in ms (-1)=50, error in (no error)=w209) -> (error out=w207:errorcluster)  [unwired: 2 out]
        }
        n91 = case shown="False" w181 {
          tunnel: w180 -> [w190 w205]
          tunnel: [w189 w205] -> w179
          tunnel: w178 -> [w194 w204]
          tunnel: [w193 w204] -> w177
          frame False {
            # "do this on first PostUI Event (happens when panel loads)"
            # "Initialize the DAQmx channel control"
            n92 = local read "digital serial cfg file"() -> (w187:string)
            n93 = local read "power measurement resource"() -> (w197:string)
            n94 = local read "acq channel"() -> (w196:string)
            n95 = Empty String/Path?(string/path=w187) -> (empty?=w192:bool)
            n96 = local write "power meas resource"(w197) -> ()
            n97 = property on="Acquisition channel" class="DAQmxName"("Value"=w196) -> ()  [unwired: 2 in, 2 out]
            n98 = case shown="True" w192 {
              tunnel: w190 -> [w199 w203]
              tunnel: [w199 w201] -> w191
              tunnel: w187 -> [w198 _]
              tunnel: [w198 w200] -> w186
              frame False {
              }
              frame True {
                n99 = call "Get Audio Settings.vi"("error in (no error)"=w203) -> ("error out"=w201:errorcluster, "audio settings"=w202:T12)  [unwired: 9 in]
                n100 = Unbundle By Name(w202) -> ("digital serial file"=w200:string)
              }
            }
            n101 = String To Path(string=w186) -> (path=w188:path)
            n102 = call "Get Display Name for Cfg file.vi"("error in (no error)"=w191, "file path"=w188) -> ("error out"=w189:errorcluster, "display string"=→"digital serial file name":string)  [unwired: 8 in]
            n103 = local write "digital serial cfg file"(w186) -> ()
            n104 = Bundle By Name(cluster=w194, "PostUI event occurred"=TRUE, "digital serial cfg file"=w188) -> (w193:T8)
          }
          frame True {
          }
        }
      }
      frame "Update Graphs" {
        # "This case will be triggered, after framework updates the User interface with result values."
        n105 = local read "channel names"() -> (w212:string[])
        n106 = control-ref of="time domain"() -> (w215:refnum<vi>)
        n107 = control-ref of="frequency domain"() -> (w211:refnum<vi>)
        n108 = local read "wfm - data"() -> (w222:dbl[])
        n109 = local read "wfm - dt"() -> (w221:dbl)
        n110 = local read "fft - data"() -> (w219:dbl[])
        n111 = local read "fft - df"() -> (w218:dbl)
        n112 = local read "fft - f0"() -> (w217:dbl)
        n113 = call "Array to Wfm (N Ch).vi"("channel names"=w212, "dt"=w221, "array"=w222) -> ("waveforms"=→"time domain":waveform(dbl)[])  [unwired: 8 in]
        n114 = call "Array to Spectra (N Ch).vi"("channel names"=w212, "df"=w218, "f0"=w217, "data"=w219) -> ("spectra"=→"frequency domain":cluster{"f0":dbl, "df":dbl, "data":dbl[]}[])  [unwired: 7 in]
        n115 = for {
          tunnel: w211 -> [w225]
          tunnel: w212 -> [_] mode=indexing
          i -> [w226]
          # "make all plots visible"
          n116 = property class="WFGraph (strict)"(reference=w225, "Active Plot"=w226, "Plot.Visible?"=TRUE ("Plot.Visible")) -> ()  [unwired: 1 in, 2 out]
        }
        n117 = for {
          tunnel: w215 -> [w228]
          tunnel: w212 -> [_] mode=indexing
          i -> [w229]
          # "make all plots visible"
          n118 = property class="WFGraph (strict)"(reference=w228, "Active Plot"=w229, "Plot.Visible?"=TRUE ("Plot.Visible")) -> ()  [unwired: 1 in, 2 out]
        }
        n119 = Array Size(array=w212) -> (size(s)=w214:i32)
        n120 = property class="WFGraph (strict)"(reference=w215, "LegNumRows"=w214, "LegScrollVis"=FALSE ("Legend:Scrollbar Visible")) -> ()  [unwired: 1 in, 2 out]
      }
      frame "Update Table" {
        # "format data for table"
        # "This case will be triggered, after framework updates the User interface with result values."
        n121 = local read "SNR units"() -> (w275:T7)
        n122 = local read "THD+N units"() -> (w287:T6)
        n123 = local read "THD units"() -> (w273:T6)
        n124 = local read "gain units"() -> (w271:T6)
        n125 = case shown="\"x/y\"" w275 {
          tunnel: ["(dB)" "(ratio)"] -> w286
          tunnel: ["%5.1f" ("initial string") "%.1f" ("initial string")] -> w269
          frame "dB", Default {
          }
          frame "x/y" {
          }
        }
        n126 = case shown="\"x/y\"" w287 {
          tunnel: ["(dB)" "(%)" "(ratio)"] -> w289
          tunnel: ["%5.1f" ("initial string") "%.3f" ("initial string") "%.6f" ("initial string")] -> w266
          frame "dB", Default {
          }
          frame "%" {
          }
          frame "x/y" {
          }
        }
        n127 = case shown="\"x/y\"" w273 {
          tunnel: ["(dB)" "(%)" "(ratio)"] -> w274
          tunnel: ["%5.1f" ("initial string") "%.3f" ("initial string") "%.6f" ("initial string")] -> w263
          frame "dB", Default {
          }
          frame "%" {
          }
          frame "x/y" {
          }
        }
        n128 = case shown="\"%\"" w271 {
          tunnel: ["(dB)" "(%)" "(ratio)"] -> w272
          tunnel: ["%5.1f" ("initial string") "%.1f" ("initial string") "%.3f" ("initial string")] -> w253
          frame "dB", Default {
          }
          frame "%" {
          }
          frame "x/y" {
          }
        }
        n129 = Concatenate Strings("SNR " ("string"), w286) -> (w283:string)
        n130 = Concatenate Strings("THD+N " ("string"), w289) -> (w282:string)
        n131 = Concatenate Strings("Gain " ("string"), w272) -> (w280:string)
        n132 = Concatenate Strings("THD " ("string"), w274) -> (w281:string)
        n133 = property on="meas table" class="Tbl (strict)"() -> ("Column Headers[]"=w236:string[])  [unwired: 2 in, 2 out]
        n134 = Replace Array Subset(array=w236, new element #1=w283, index #1=5 ("index"), new element #2=w282, index #2=6 ("index"), new element #3=w281, index #3=7 ("index"), new element #4=w280, index #4=9 ("index")) -> (w284:string[])
        n135 = property on="meas table" class="Tbl (strict)"("Column Headers[]"=w284) -> ()  [unwired: 2 in, 2 out]
        n136 = local read "amplitude (Vrms)"() -> (w248:dbl[])
        n137 = local read "amplitude (dBFS)"() -> (w245:dbl[])
        n138 = local read "frequency (Hz)"() -> (w251:dbl[])
        n139 = local read "phase (deg)"() -> (w241:dbl[])
        n140 = local read "THD+N"() -> (w268:dbl[])
        n141 = local read "THD"() -> (w265:dbl[])
        n142 = local read "SNR"() -> (w270:dbl[])
        n143 = local read "channel names"() -> (w233:string[])
        n144 = for {
          tunnel: [w306] -> w250 mode=indexing
          tunnel: w251 -> [w305] mode=indexing
          tunnel: "%.3f" ("initial string") -> [w304]
          n145 = Format Into String(format string=w304, w305) -> (resulting string=w306:string)  [unwired: 2 in, 1 out]
        }
        n146 = for {
          tunnel: [w303] -> w247 mode=indexing
          tunnel: w248 -> [w302] mode=indexing
          tunnel: "%.3f" ("initial string") -> [w301]
          n147 = Format Into String(format string=w301, w302) -> (resulting string=w303:string)  [unwired: 2 in, 1 out]
        }
        n148 = for {
          tunnel: [w300] -> w244 mode=indexing
          tunnel: w245 -> [w299] mode=indexing
          tunnel: "%.3f" ("initial string") -> [w298]
          n149 = Format Into String(format string=w298, w299) -> (resulting string=w300:string)  [unwired: 2 in, 1 out]
        }
        n150 = for {
          tunnel: [w321] -> w264 mode=indexing
          tunnel: w265 -> [w320] mode=indexing
          tunnel: w263 -> [w319]
          n151 = Format Into String(format string=w319, w320) -> (resulting string=w321:string)  [unwired: 2 in, 1 out]
        }
        n152 = for {
          tunnel: [w327] -> w259 mode=indexing
          tunnel: w270 -> [w326] mode=indexing
          tunnel: w269 -> [w325]
          n153 = Format Into String(format string=w325, w326) -> (resulting string=w327:string)  [unwired: 2 in, 1 out]
        }
        n154 = for {
          tunnel: [w324] -> w267 mode=indexing
          tunnel: w268 -> [w323] mode=indexing
          tunnel: w266 -> [w322]
          n155 = Format Into String(format string=w322, w323) -> (resulting string=w324:string)  [unwired: 2 in, 1 out]
        }
        n156 = for {
          tunnel: [w297] -> w242 mode=indexing
          tunnel: w241 -> [w296] mode=indexing
          tunnel: "%.3f" ("initial string") -> [w295]
          n157 = Format Into String(format string=w295, w296) -> (resulting string=w297:string)  [unwired: 2 in, 1 out]
        }
        n158 = local read "dynamic range (dB)"() -> (w261:dbl[])
        n159 = local read "output power (W)"() -> (w257:dbl[])
        n160 = local read "SFDR (dBc)"() -> (w255:dbl[])
        n161 = local read "gain"() -> (w254:dbl[])
        n162 = for {
          tunnel: [w318] -> w260 mode=indexing
          tunnel: w261 -> [w317] mode=indexing
          tunnel: "%5.1f" ("initial string") -> [w316]
          n163 = Format Into String(format string=w316, w317) -> (resulting string=w318:string)  [unwired: 2 in, 1 out]
        }
        n164 = for {
          tunnel: [w309] -> w240 mode=indexing
          tunnel: w254 -> [w308] mode=indexing
          tunnel: w253 -> [w307]
          n165 = Format Into String(format string=w307, w308) -> (resulting string=w309:string)  [unwired: 2 in, 1 out]
        }
        n166 = for {
          tunnel: [w312] -> w239 mode=indexing
          tunnel: w255 -> [w311] mode=indexing
          tunnel: "%5.1f" ("initial string") -> [w310]
          n167 = Format Into String(format string=w310, w311) -> (resulting string=w312:string)  [unwired: 2 in, 1 out]
        }
        n168 = for {
          tunnel: [w315] -> w238 mode=indexing
          tunnel: w257 -> [w314] mode=indexing
          tunnel: "%.3f" ("initial string") -> [w313]
          n169 = Format Into String(format string=w313, w314) -> (resulting string=w315:string)  [unwired: 2 in, 1 out]
        }
        n170 = Build Array(w233, w250, w247, w244, w242, w259, w267, w264, w260, w240, w239, w238) -> (w237:string[][])
        n171 = Transpose 2D Array(2D array=w237) -> (transposed array=w234:string[][])
        "meas table" <- w234
        n172 = flat-sequence {
          tunnel: [w294] -> w235
          tunnel: w234 -> [_]
          tunnel: w231 -> [w292]
          frame #0 {
            n173 = control-ref of="meas table"() -> (w293:refnum<vi>)
            n174 = call "Autosize Columns (Table).vi"("error in (no error)"=w292, "table"=w293) -> ("error out"=w294:errorcluster)  [unwired: 9 in]
          }
        }
      }
      frame "Exit" {
        # "This case is triggered to close the User Interface from framework"
        n175 = Flush Queue(queue=w355, error in (no error)=w357) -> (queue out=w354:refnum<queue>, error out=w353:errorcluster)  [unwired: 1 out]
        n176 = Release Queue(queue=w354, force destroy? (F)=TRUE, error in (no error)=w353) -> (error out=w352:errorcluster)  [unwired: 2 out]
      }
      frame "Handle Error" {
      }
    }
    n177 = call <vilib>:"Simple Error Handler.vi"("error in (no error)"=w18) -> ()  [unwired: 4 in, 5 out]
  }
